vi "VM - 1D Array of Strings.vi"(6 "global? (F)":bool, 7 "VC Handle":T3=-1, 8 "error in":errorcluster, 9 "cmd":T2(ring)=enum."get value", 10 "value in":string[](array[string]), 11 "name_spec":string) -> (0 "error out":errorcluster, 1 "err code":T1 items=["No error", "Invalid variable type", "Variable not found", "Variable already exists", "Invalid context handle", "Input error", "Invalid data format", "No history attached", "History already attached", "Invalid history parameters", "Wrong variable name", "Wrong alias name", "Non-unique alias", "Alias not found", "No alias associated", "Alias already associated", "Wrong context name", "Non-unique context name", "Context name not found", "Invalid parameter", "Generic error", "Memory Full", "Unrecognized LV error", "Unknown error code"], 2 "value out":string[](array[string]), 3 "dup name_spec":string, 4 "global out":bool, 5 "dup VC Handle":T3=-1)   [LabVIEW 2021]
doc: "This VI manages variables of the <b>1D Array of Strings</b> data type. Refer to the VI help for more details.\n\n<b>VC Handle</b> specifies the handle of the variable context. This input is ignored if the <b>name_spec</b> control refers to a variable by an alias during 'get value', 'set value', and 'destroy' actions or if the action is 'create' and <b>global?</b> is TRUE.\n\n<b>name_spec</b> is the name specifier of the desired variable. Usually, it is merely a variable name; however, its generic format is '[name][=alias]', where either 'name' or '=alias' can be omitted but not both.\n\n<b>cmd</b> control specifies the action to be performed on the variable. Possible actions are 'create', 'destroy', 'get value', and 'set value'.\n\n<b>value in</b> control specifies the value to be written to the variable; it is only used during 'set value' or 'create' actions. <b>value out</b> indicator returns the value that has been read from the variable.\n\n<b>global?</b> control, if TRUE, enables access to global variables. For 'create' and 'destroy' actions, it causes the VI to ignore <b>VC Handle</b> and operate on a global variable. For 'get value' and 'set value' actions, it allows the VI to operate on a global variable if the specified variable name is not found in the context specified by <b>VC Handle</b>.\n\n<b>global out</b> indicator returns TRUE if an action has been performed on a global variable.\n\n<b>err code</b> indicator returns a VarMan Engine error code.\n\n::: CalcExpress Toolkit :::\nCopyright (c) 2000-2026 Konstantin Shifershteyn. All rights reserved."
uses:
  cetypes.llb/VarMan Variable Context Handle.ctl
  cetypes.llb/VarMan Error Code.ctl
  cersrc/celveng32.dll
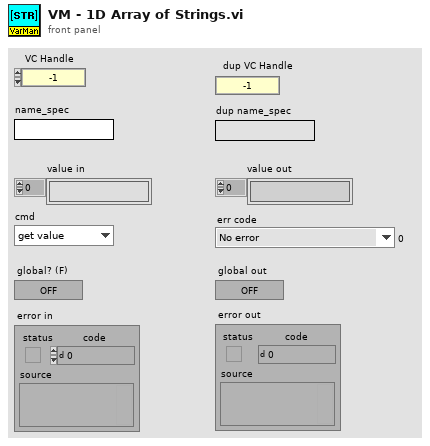
[diagram p1: front panel]
types:
  T1 = typedef "VarMan Error Code.ctl" = u16
  T2 = enum16{"create", "destroy", "set value", "get value"}
  T3 = typedef "VarMan Variable Context Handle.ctl" = i32
  T4 = enum32{"String", "DBL Number", "identifier", "1D Array of DBL", "2D Array of DBL", "CDB Number", "1D Array of CDB", "2D Array of CDB", "1D Array of String", "2D Array of String", "Unknown data type"}
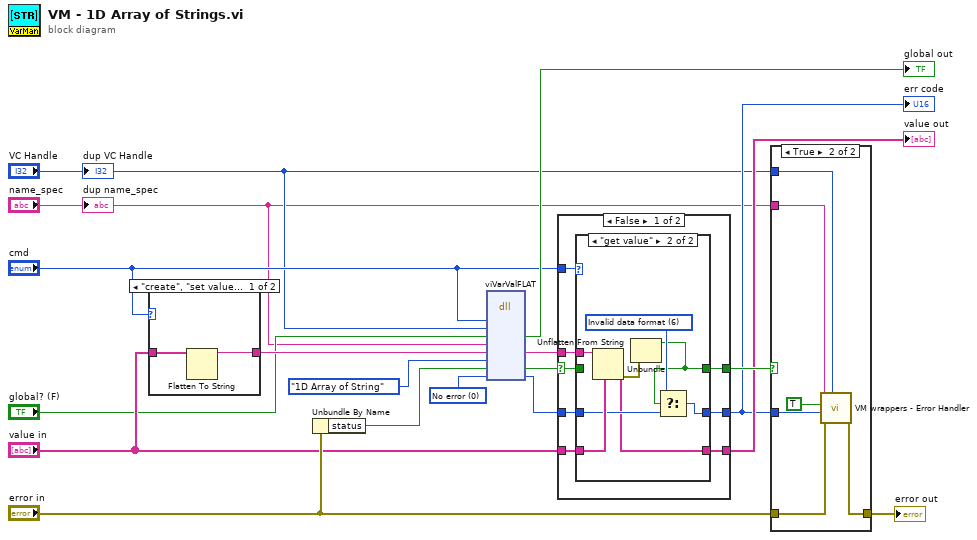
[diagram p0: block diagram]
diagram:
  w11 = T1 0 items=["No error", "Invalid variable type", "Variable not found", "Variable already exists", "Invalid context handle", "Input error", "Invalid data format", "No history attached", "History already attached", "Invalid history parameters", "Wrong variable name", "Wrong alias name", "Non-unique alias", "Alias not found", "No alias associated", "Alias already associated", "Wrong context name", "Non-unique context name", "Context name not found", "Invalid parameter", "Generic error", "Memory Full", "Unrecognized LV error", "Unknown error code"] ("VarMan error")
  n1 = case shown="\"create\", \"set value\"" "cmd" {
    tunnel: [w20 _] -> w16
    tunnel: "value in" -> [w19 _]
    frame "create", "set value" {
      n2 = Flatten To String(anything=w19) -> (data string=w20:string)  [unwired: 3 in, 2 out]
    }
    frame Default {
    }
  }
  n3 = Unbundle By Name("error in") -> ("status"=w17:bool)
  n4 = dll-call lib="C:/LV Projects/CalcExpress 40 LV2021/vi.lib/addons/CalcExpress/cersrc/celveng*.dll" fn="viVarValFLAT"("cmd"="cmd", "vch"="VC Handle", "gbl"="global? (F)", "name"="name_spec", w16, "type"=T4."1D Array of String" ("data type"), w17, "errc"=w11) -> ("gbl"=→"global out":bool, w13:string, w14:bool, "errc"=w12:T1)  [unwired: 8 in, 2 out]
  n5 = case shown="False" w14 {
    selector: w14 -> [w22 w42]
    tunnel: w13 -> [w27 _]
    tunnel: "cmd" -> [w28 _]
    tunnel: [w25 w42] -> w18
    tunnel: "value in" -> [w26 w40]
    tunnel: w12 -> [w24 w41]
    tunnel: [w23 w41] -> w9
    tunnel: [w21 w40] -> w10
    frame False {
      n6 = case shown="\"get value\"" w28 {
        tunnel: w27 -> [_ w39]
        tunnel: w26 -> [w29 w38]
        tunnel: [w30 w32] -> w25
        tunnel: w24 -> [w31 w37]
        tunnel: [w31 w35] -> w23
        tunnel: w22 -> [w30 _]
        tunnel: [w29 w34] -> w21
        frame Default {
        }
        frame "get value" {
          w36 = T1 6 items=["No error", "Invalid variable type", "Variable not found", "Variable already exists", "Invalid context handle", "Input error", "Invalid data format", "No history attached", "History already attached", "Invalid history parameters", "Wrong variable name", "Wrong alias name", "Non-unique alias", "Alias not found", "No alias associated", "Alias already associated", "Wrong context name", "Non-unique context name", "Context name not found", "Invalid parameter", "Generic error", "Unknown error code"] ("VarMan error")
          n7 = Unflatten From String(type=w38, binary string=w39) -> (value=w34:string[], error out=w33:errorcluster)  [unwired: 3 in, 1 out]
          n8 = Unbundle(w33) -> ("status"=w32:bool)  [unwired: 2 out]
          n9 = Select(t=w36, s=w32, f=w37) -> (s? t:f=w35:T1)
        }
      }
    }
    frame True {
    }
  }
  "value out" <- w10
  "err code" <- w9
  n10 = case shown="True" w18 {
    tunnel: [w43 w49] -> w7
    tunnel: "error in" -> [w43 w48]
    tunnel: w9 -> [_ w46]
    tunnel: "name_spec" -> [_ w47]
    tunnel: "VC Handle" -> [_ w44]
    frame False {
    }
    frame True {
      n11 = call "VM wrappers - Error Handler.vi"("VC Handle"=w44, "error before"=w48, "VarMan error"=w46, "show name spec (F)"=TRUE, "name spec"=w47) -> ("error out"=w49:errorcluster)  [unwired: 5 in, 1 out]
    }
  }
  "error out" <- w7
  "dup VC Handle" <- "VC Handle"
  "dup name_spec" <- "name_spec"
